vi "Batch Averager Scaled.vi"() -> ()   [LabVIEW 2026]
doc: "Round5 edit-loop demo: the round4 Batch Averager state machine patched by adding one Scale control (uid 105) and one Multiply node (uid 610) in the Accumulate frame. Patch applied to the handwritten AIXML source (batch-averager.aixml.xml from round4), then regenerated. Semantics: each item is multiplied by Scale before being added to the sum, so Average = Scale * mean(Items)."
panel:
  out "Log":string
  out "Average":dbl
  out "Items Processed":i32
  out "Sum":dbl
  out "Final State":T1(ring)
  in  "Scale":dbl=1.0
  in  "Items":dbl[](array[numeric])=[1.5, 2.5, 3.5, 4.5]
  in  "Initial State":T1(ring)
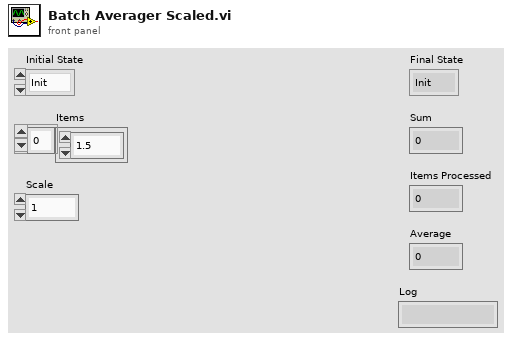
[diagram p1: front panel]
types:
  T1 = enum16{"Init", "Load", "Accumulate", "Report", "Stop"}
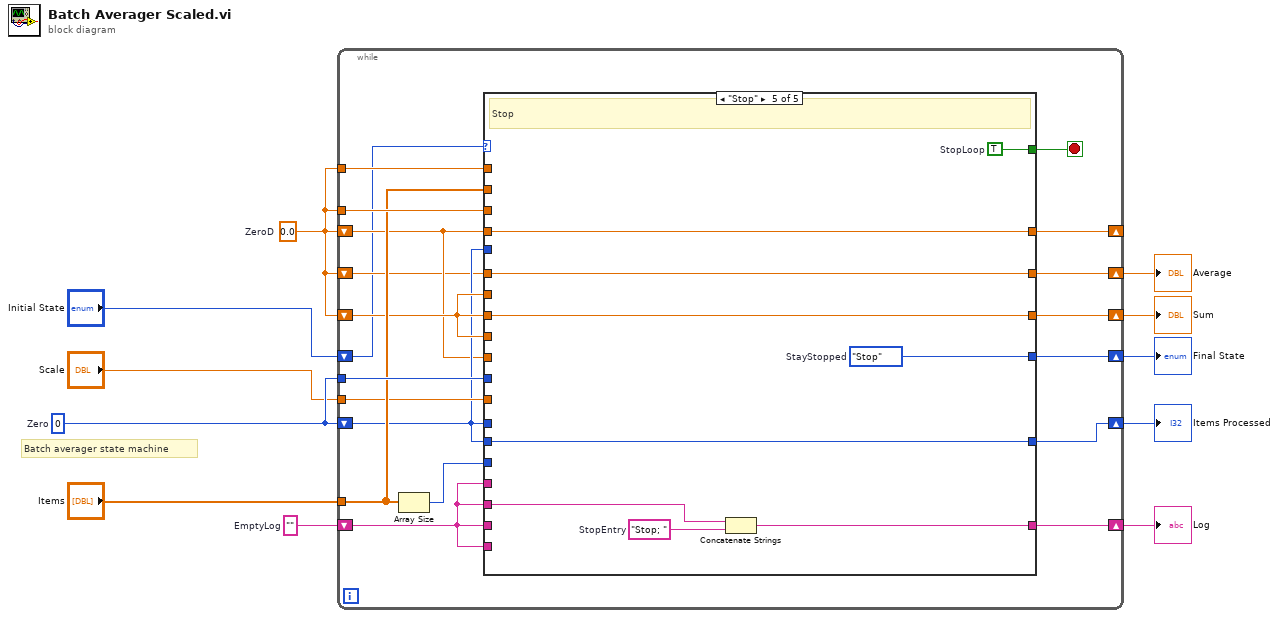
[diagram p0: block diagram]
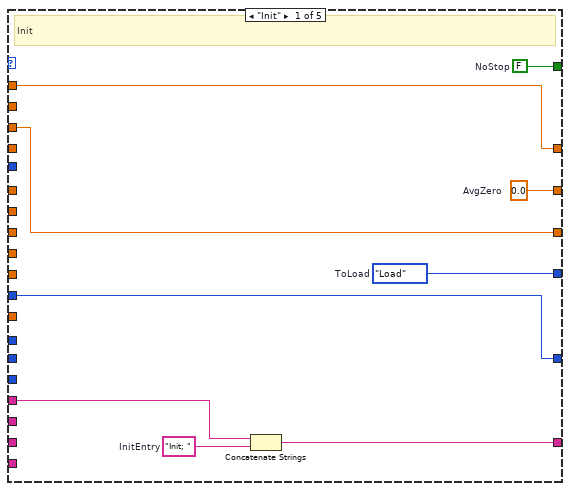
[diagram p2: hidden frame]
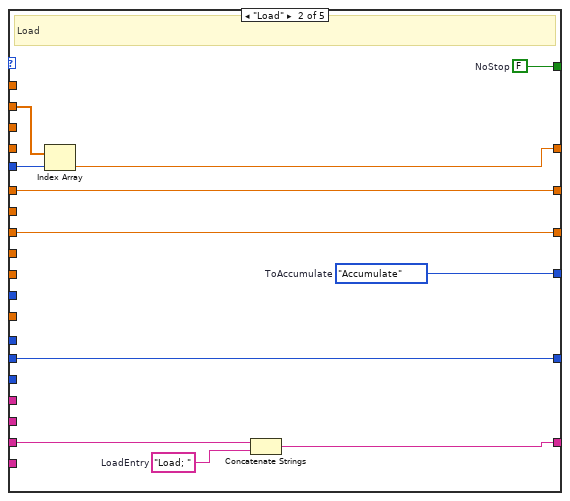
[diagram p3: hidden frame]
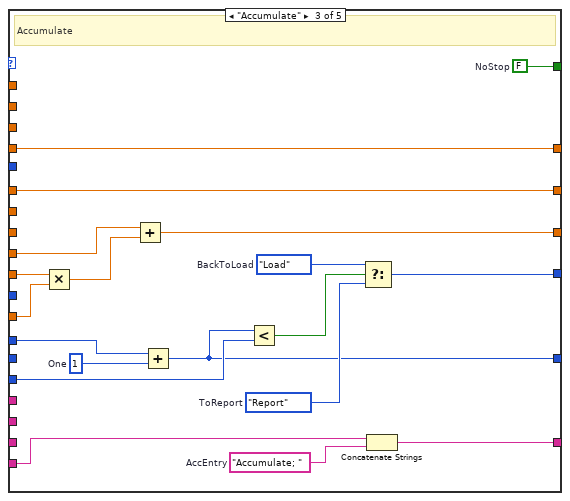
[diagram p4: hidden frame]
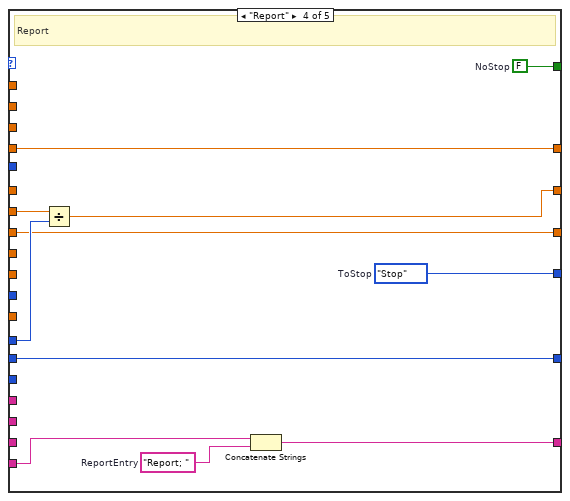
[diagram p5: hidden frame]
diagram:
  w9 = ""  # EmptyLog
  w7 = 0.0  # ZeroD
  w8 = 0  # Zero
  # "Batch averager state machine"
  n1 = while {
    tunnel: "Items" -> [w20]
    shift-right: [w30] -> w5
    shift-left: "Initial State" -> [w12]
    shift-right: [w28] -> w4
    shift-left: w7 -> [w16]
    shift-right: [w27] -> w3
    shift-left: w8 -> [w15]
    shift-right: [w26] -> _
    shift-left: w7 -> [w14]
    shift-right: [w25] -> w1
    shift-left: w9 -> [w17]
    shift-right: [w24] -> w2
    shift-left: w7 -> [w13]
    tunnel: w7 -> [w23]
    tunnel: w8 -> [w22]
    tunnel: w7 -> [w21]
    tunnel: "Scale" -> [w19]
    stop <- w29 stop-if-true
    n2 = Array Size(array=w20) -> (size(s)=w18:i32)
    n3 = case shown="\"Stop\"" w12 {
      tunnel: [w39 w48 w59 w78 w89] -> w30
      tunnel: [w38 w47 w58 w77 w88] -> w29
      tunnel: [w34 w43 w54 w73 w84] -> w28
      tunnel: [w33 w42 w53 w72 w83] -> w27
      tunnel: [w32 w41 w52 w71 w82] -> w26
      tunnel: [w35 w44 w55 w74 w85] -> w25
      tunnel: [w31 w40 w51 w70 w81] -> w24
      tunnel: w17 -> [w37 _ _ _ _]
      tunnel: w23 -> [w34 _ _ _ _]
      tunnel: w22 -> [w33 _ _ _ _]
      tunnel: w21 -> [w32 _ _ _ _]
      tunnel: w20 -> [_ w50 _ _ _]
      tunnel: w15 -> [_ w49 _ _ _]
      tunnel: w17 -> [_ w46 _ _ _]
      tunnel: w14 -> [_ _ w69 _ _]
      tunnel: w19 -> [_ _ w68 _ _]
      tunnel: w16 -> [_ _ w67 _ _]
      tunnel: w18 -> [_ _ w63 _ _]
      tunnel: w16 -> [_ _ _ w80 _]
      tunnel: w15 -> [_ _ w65 w79 _]
      tunnel: w17 -> [_ _ w57 w76 _]
      tunnel: w17 -> [_ _ _ _ w87]
      tunnel: w16 -> [_ w43 _ w73 w84]
      tunnel: w15 -> [_ w42 _ w72 w83]
      tunnel: w14 -> [_ _ w52 w71 w82]
      tunnel: w13 -> [_ w40 w51 _ w81]
      frame "Init" {
        w31 = 0.0  # AvgZero
        w36 = "Init; "  # InitEntry
        w38 = FALSE  # NoStop
        w39 = T1."Load"  # ToLoad
        # "Init"
        n4 = Concatenate Strings(w37, w36) -> (w35:string)
      }
      frame "Load" {
        w45 = "Load; "  # LoadEntry
        w47 = FALSE  # NoStop
        w48 = T1."Accumulate"  # ToAccumulate
        # "Load"
        n5 = Index Array(array=w50, index=w49) -> (element=w41:dbl)
        n6 = Concatenate Strings(w46, w45) -> (w44:string)
      }
      frame "Accumulate" {
        w56 = "Accumulate; "  # AccEntry
        w58 = FALSE  # NoStop
        w60 = T1."Report"  # ToReport
        w62 = T1."Load"  # BackToLoad
        w64 = 1  # One
        # "Accumulate"
        n7 = Multiply(x=w69, y=w68) -> (x*y=w66:dbl)
        n8 = Add(x=w67, y=w66) -> (x+y=w54:dbl)
        n9 = Add(x=w65, y=w64) -> (x+y=w53:i32)
        n10 = Less?(x=w53, y=w63) -> (x < y?=w61:bool)
        n11 = Select(t=w62, s=w61, f=w60) -> (s? t:f=w59:T1)
        n12 = Concatenate Strings(w57, w56) -> (w55:string)
      }
      frame "Report" {
        w75 = "Report; "  # ReportEntry
        w77 = FALSE  # NoStop
        w78 = T1."Stop"  # ToStop
        # "Report"
        n13 = Divide(x=w80, y=w79) -> (x/y=w70:dbl)
        n14 = Concatenate Strings(w76, w75) -> (w74:string)
      }
      frame "Stop" {
        w86 = "Stop; "  # StopEntry
        w88 = TRUE  # StopLoop
        w89 = T1."Stop"  # StayStopped
        # "Stop"
        n15 = Concatenate Strings(w87, w86) -> (w85:string)
      }
    }
  }
  "Final State" <- w5
  "Sum" <- w4
  "Items Processed" <- w3
  "Average" <- w2
  "Log" <- w1
